vi "NI32LV2612f2ASD3_Untitled 4.vi"() -> ()   [LabVIEW 2026]
panel:
  out "Array 2":dbl[](array[numeric])
  out "Array":dbl[](array[numeric])
  in  "array":dbl[](array[numeric])
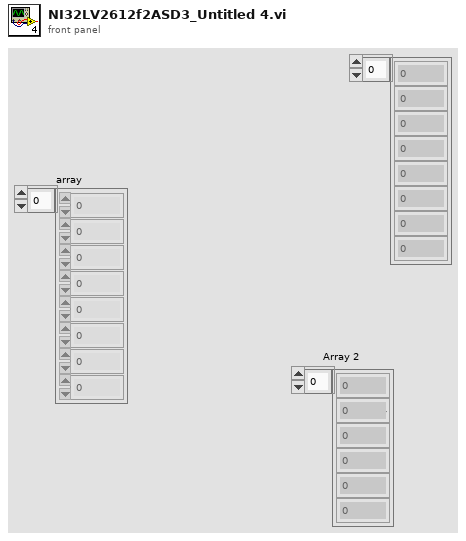
[diagram p1: front panel]
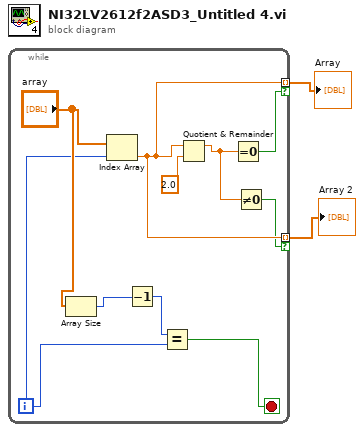
[diagram p0: block diagram]
diagram:
  n1 = while {
    tunnel: [w5] -> w2 mode=indexing if=w7
    tunnel: [w5] -> w1 mode=indexing if=w4
    i -> [w9]
    stop <- w6 stop-if-true
    n2 = Array Size(array="array") -> (size(s)=w12:i32)
    n3 = Index Array "Index Array"(array="array", index=w9) -> (element=w5:dbl)
    n4 = Decrement(x=w12) -> (x-1=w11:i32)
    n5 = Equal?(x=w11, y=w9) -> (x = y?=w6:bool)
    n6 = Quotient & Remainder(x=w5, y=2.0) -> (x-y*floor(x/y)=w3:dbl)  [unwired: 1 out]
    n7 = Equal To 0?(x=w3) -> (x = 0?=w7:bool)
    n8 = Not Equal To 0?(x=w3) -> (x != 0?=w4:bool)
  }
  "Array" <- w2
  "Array 2" <- w1
